vi "Easy Read XML File.vi"(8 "error in (no error)":errorcluster, 9 "LabVIEW Data (Type)":variant, 11 "XML File Path":path) -> (0 "error out":errorcluster, 2 "LabVIEW Data":variant, 3 "XML File Path (duplicate)":path)   [LabVIEW 2011]
doc: "Reads and parses data from an XML file (specified by the <B>XML File Path</B> input), converting it into <B>LabVIEW Data</B>, based on the <B>LabVIEW Data (Type)</B> argument. Use the <B>Variant to Data</B> function to convert the output variant <B>LabVIEW Data</B> to the desired data type."
uses:
  <userlib>/_OpenG.lib/lvdata/lvdata.llb/Type Descriptor Enumeration__ogtk.ctl
panel:
  # "JKI EasyXML Toolkit for LabVIEW\nhttp://jki.net/easyxml\nCopyright (C) 2007-2016, JKI <info@jki.net>\nALL RIGHTS RESERVED"
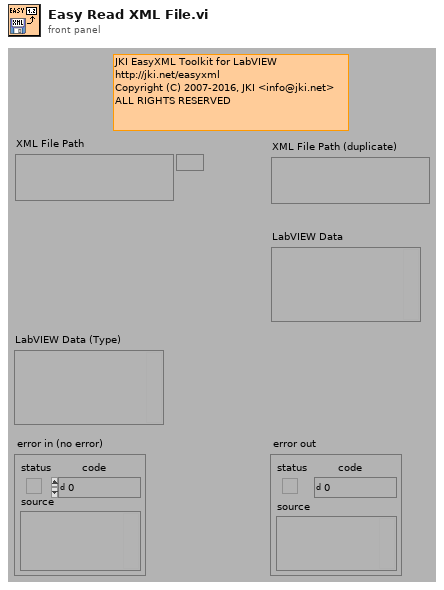
[diagram p1: front panel]
types:
  T1 = typedef "Type Descriptor Enumeration__ogtk.ctl" = enum8{"<Null>", "I8", "I16", "I32", "I64", "U8", "U16", "U32", "U64", "SGL", "DBL", "EXT", "CSG", "CDB", "CXT", "0x0F", "0x10", "0x11", "0x12", "0x13", "0x14", "Enum U8", "Enum U16", "Enum U32", "Enum U64", "SGL PQ", "DBL PQ", "EXT PQ", "CSG PQ", "CDB PQ", "CXT PQ", "0x1F", "0x20", "Boolean", "0x22", "0x23", "0x24", "0x25", "0x26", "0x27", "0x28", "0x29", "0x2A", "0x2B", "0x2C", "0x2D", "0x2E", "0x2F", "String", "0x31", "Path", "Pict", "0x34", "0x35", "0x36", "DAQ", "0x38", "0x39", "0x3A", "0x3B", "0x3C", "0x3D", "0x3E", "0x3F", "Array", "0x41", "0x42", "0x43", "0x44", "0x45", "0x46", "0x47", "0x48", "0x49", "0x4A", "0x4B", "0x4C", "0x4D", "0x4E", "0x4F", "Cluster", "0x51", "0x52", "Variant", "Waveform", "0x55", "0x56", "0x57", "0x58", "0x59", "0x5A", "0x5B", "0x5C", "0x5D", "0x5E", "0x5F", "0x60", "0x61", "0x62", "0x63", "0x64", "0x65", "0x66", "0x67", "0x68", "0x69", "0x6A", "0x6B", "0x6C", "0x6D", "0x6E", "0x6F", "Refnum"}
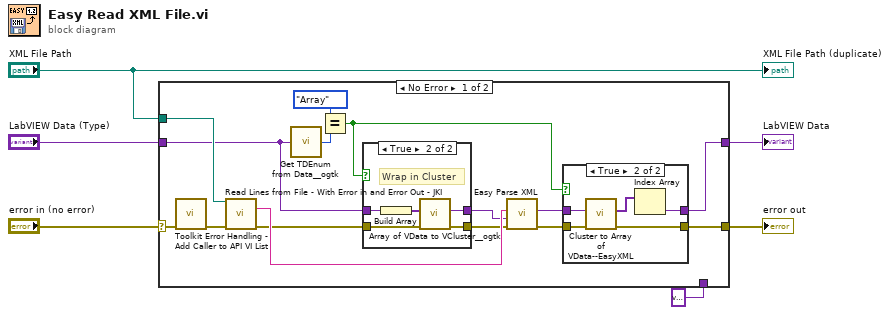
[diagram p0: block diagram]
diagram:
  n1 = case shown="No Error" "error in (no error)" {
    selector: "error in (no error)" -> [w8 w37]
    tunnel: [w11 w37] -> w5
    tunnel: "XML File Path" -> [w21 _]
    tunnel: "LabVIEW Data (Type)" -> [w15 _]
    tunnel: [w9 w36] -> w2
    tunnel: variant ("LabVIEW Data") -> [_ w36]
    frame No Error {
      n2 = call "Toolkit Error Handling - Add Caller to API VI List.vi"("error in"=w8) -> ("error out"=w7:errorcluster)  [unwired: 10 in]
      n3 = call "Read Lines from File - With Error in and Error Out - JKI.vi"("file path (dialog if empty)"=w21, "error in (no error)"=w7) -> ("line string"=w20:string, "error out"=w17:errorcluster)  [unwired: 9 in, 3 out]
      n4 = call <userlib>:"Get TDEnum from Data__ogtk.vi"("Data"=w15) -> ("Type Descriptor Enumeration"=w19:T1)  [unwired: 4 in]
      n5 = Equal?(x=Type_Descriptor_Enumeration__ogtk."Array" ("Type Descriptor Enumeration"), y=w19) -> (x = y?=w10:bool)
      n6 = case shown="True" w10 {
        tunnel: w17 -> [w30 w34]
        tunnel: [w30 w33] -> w16
        tunnel: w15 -> [w29 w32]
        tunnel: [w29 w31] -> w14
        frame False {
        }
        frame True {
          # "Wrap in Cluster"
          n7 = Build Array(w32) -> (w35:variant[])
          n8 = call <userlib>:"Array of VData to VCluster__ogtk.vi"("error in (no error)"=w34, "Array"=w35) -> ("error out"=w33:errorcluster, "VCluster"=w31:variant)  [unwired: 8 in]
        }
      }
      n9 = call "Easy Parse XML.vi"("error in (no error)"=w16, "LabVIEW Data (Type)"=w14, "XML String"=w20) -> ("error out"=w12:errorcluster, "LabVIEW Data"=w13:variant)  [unwired: 7 in]
      n10 = case shown="True" w10 {
        tunnel: w13 -> [w22 w28]
        tunnel: w12 -> [w23 w27]
        tunnel: [w23 w26] -> w11
        tunnel: [w22 w24] -> w9
        frame False {
        }
        frame True {
          n11 = call "Cluster to Array of VData--EasyXML.vi"("error in (no error)"=w27, "Cluster"=w28) -> ("error out"=w26:errorcluster, "Array of VData"=w25:variant[])  [unwired: 8 in]
          n12 = Index Array(array=w25) -> (element=w24:variant)  [unwired: 1 in]
        }
      }
    }
    frame Error {
    }
  }
  "error out" <- w5
  "LabVIEW Data" <- w2
  "XML File Path (duplicate)" <- "XML File Path"
